vi "CIMfpgaVI.vi"() -> ()   [LabVIEW 2016]
uses:
  Controls/StatesCIM.ctl
  Controls/srcmODE.ctl
  <vilib>/rvi/eio/common/nirviEmuClasses.ctl
  <vilib>/rvi/Emulation/niFpgaGetClockAttributes.vi
  <vilib>/rvi/Emulation/niFpgaSctlEmulationGetInTimedLoop.vi
  <vilib>/rvi/Emulation/niFpgaEmulationReportErrorSimple.vi
  <vilib>/rvi/Emulation/niFpgaProcessEmulError.vi
  <vilib>/rvi/Emulation/niFpgaCriticalErrorInLSC.vi
  <vilib>/rvi/occurrence/nirviWaitOnOccurrenceBase.vi
  <vilib>/rvi/Emulation/niFpgaEmulationIsFPGAContextNoSignature.vi
  <vilib>/rvi/errors/niFpgaSetErrorForExecOnDevCompSimple.vi
  <vilib>/rvi/eio/common/nirviEmuReportErrorAndStop.vi
  <vilib>/rvi/DataTransferAndStorage/Container/Common/niFpgaContainerGetUniqueNameForEmu.vi
  <vilib>/rvi/FIFO/Fifo_Resource/nirvififoEmulationSetSize.vi
  <vilib>/rvi/FIFO/Fifo_Resource/nirviFifoEmulationQueueMgr.vi
  <instcachedir>/0/nirviFifoEmulationQueueMgr_E5CAEC123FF24DC58D834DCA3CDAA9B5.lvgen/nirviFifoEmulationQueueMgr_E5CAEC123FF24DC58D834DCA3CDAA9B5_002.vi
  <vilib>/Utility/error.llb/Clear Errors.vi
  <vilib>/rvi/FIFO/Fifo_Resource/nirvififoEmulationCreateLock.vi
  <vilib>/rvi/FIFO/Fifo_Resource/nirvififoEmulationObtainLock.vi
  <vilib>/rvi/FIFO/Fifo_Resource/nirvififoEmulationReleaseLock.vi
  <vilib>/rvi/errors/nirviReportUnexpectedCaseInternalError.vi
  <vilib>/rvi/errors/nirviReportUnexpectedCaseInternalError (U32).vi
  <vilib>/rvi/eio/common/nirviEmuTemplateMethod_noerrors.vi
  <vilib>/rvi/eio/common/nirviEmuTemplateMethod_errors.vi
  <instcachedir>/0/nirviFifoEmulationQueueMgr_E5CAEC123FF24DC58D834DCA3CDAA9B5.lvgen/nirviFifoEmulationQueueMgr_E5CAEC123FF24DC58D834DCA3CDAA9B5_001.vi
  <vilib>/rvi/FIFO/Fifo_Resource/nirvififoEmulationDetermineInputValidOut.vi
  <vilib>/rvi/eio/common/nirviEmuTemplatePropertyGet_errors.vi
  <vilib>/rvi/Memory/Memory_Emulation/niFpgaMemoryEmulationCacheClearOnFirstRun.vi
  <vilib>/rvi/Memory/Memory_Emulation/nirvimemoryEmulationManagerCache_MakeExclusive.vi
  <vilib>/rvi/Memory/Memory_Emulation/niFpgaMemoryEmulationValidateCache.vi
  <vilib>/rvi/Memory/Memory_Emulation/nirvimemoryEmulationManagerCache_InsertValue.vi
  <vilib>/rvi/Memory/Memory_Emulation/nirvimemoryEmulationManagerCache_ReleaseExclusive.vi
  <vilib>/rvi/Memory/Memory_Emulation/nirvimemoryEmulationManagerCache_GetValue.vi
  <vilib>/rvi/Memory/Memory_Emulation/nirvimemoryEmulationManagerCache_SetValue.vi
  <vilib>/rvi/DataTransferAndStorage/Container/XNode/niFpgaContainer.xnode
  <vilib>/rvi/FIFO/Fifo_Resource/nirvififoEmulationRead.vi
  <vilib>/rvi/FXPMathLib/FxpMul/XNode/nifxpmath_Multiplier.xnode
  <vilib>/eio/EIOGrowableMethodNode/genericMethod/EIOGrowableMethodNode.xnode
  <vilib>/rvi/eio/nirviEIOMethodImplementation/nirviEIOMethodImplementation.xnode
  <vilib>/rvi/eio/nirviErrorMerge/nirviErrorMerge.xnode
  <vilib>/rvi/FIFO/Fifo_Resource/nirvififoEmulationWrite.vi
  <vilib>/eio/EIONode/EIONode.xnode
  <vilib>/eio/EIOPropertyNode/EIOPropertyNode.xnode
  <vilib>/eio/EIOMethodNode/EIOMethodNode.xnode
  <vilib>/rvi/DataTransferAndStorage/Register/Emulation/niFpgaRegisterEmulation.vi
  <vilib>/rvi/eio/common/nirviEmuTemplatePropertyGet_noerrors.vi
  <vilib>/rvi/eio/common/nirviEmuTemplatePropertySet_errors.vi
  <vilib>/rvi/eio/common/nirviEmuTemplatePropertySet_noerrors.vi
  <vilib>/rvi/FXPMathLib/sim/FxpSim.dll
panel:
  out "State Set":T1
  out "ACCT current":fxp<+/-,24,5>
  out "Vmon current":fxp<+/-,24,5>
  out "ACCTThr_readback":fxp<+/-,24,5>=5.5
  out "VMONThr_readback":fxp<+/-,24,5>=-3.0
  out "VMONOff_readback":fxp<+/-,24,5>=-1.0
  out "DUTY Bad Cycles":u32
  out "acct gateon":fxp<+/-,24,5>
  out "vmon gateon":fxp<+/-,24,5>
  out "Modules error":errorcluster
  out "State Diag":T1
  out "VMon Diag":fxp<+/-,24,5>
  out "ACCT Diag":fxp<+/-,24,5>
  out "FBIs":u32
  out "Faraday Diag":bool
  out "C.GATE Diag":bool
  out "Duty Diag":bool=TRUE
  out "Pulse Diag":bool=TRUE
  out "AQ DI24V 2":u32
  out "DI24V LOOP TICKS":u8 caption="Data loop time (usec)"
  out "Timed Out? 5":bool
  out "Timed Out? 6":bool
  out "Timed Out? 7":bool
  in  "DI24V timeout":i32=40
  in  "DI24V sample period (ticks)":u32=40
  out "SRCDuty":fxp<+,32,32>=20.0
  out "SRCPulse":u32=120200
  out "SRCMode":T2
  in  "RESET":bool
  in  "TTL sample period (ticks)":u32=20
  in  "TTL timeout":i32=40
  out "ANALOG LOOP TICKS 2":u8 caption="Data loop time (usec)"
  out "DITTL LOOP TICKS":u8 caption="Data loop time (usec)"
  out "FBI LOOP TICKS":u8 caption="Data loop time (usec)"
  out "Timed Out? 10":bool
  out "Timed Out? 9":bool
  out "DUTY Loop time (tick)":u32
  out "acct gateoff":fxp<+/-,24,5>
  out "Vmon gateoff":fxp<+/-,24,5>
  out "chopper gate":bool
  out "Faraday":bool
  out "chopper OK":bool
  out "acct prearm":fxp<+/-,24,5>
  out "vmon prearm":fxp<+/-,24,5>
  out "STM Loop time (tick)":u32
  out "Timed Out? 8":bool
  out "Timed Out? 2":bool
  out "Timed Out?":bool
  in  "AI sample period (usec)":u32=1
  out "DUTY CYCLING":u32
  out "BULCE AQ GRANDE":i32
  out "DO24V":u32
  out "AQ DITTL":u32
  out "AQ ANALOG STATUS":u32
  out "AQ ANALOG PULSOS":u32
  out "Duty Waiting?":bool
  out "Aquisition Waiting?":bool
  in  "AI Timeout":i32=400
  out "AQ ANALOG AI01":u32
  out "A. READ timeout":bool
  out "current state":T1
  out "State machine iterations":u32
  out "config":i32
  in  "ACCTThr":fxp<+/-,24,5>=5.5
  in  "VMONThr":fxp<+/-,24,5>=-3.0
  in  "GATETFall (us)":u8=15
  in  "GATETRise (us)":u8=15
  in  "VMONOff":fxp<+/-,24,5>=-1.0
  out "FBI":bool
  out "cRIOModulesOK":bool
  out "Mod1Present 4":bool
  out "Mod1Present 3":bool
  out "Mod1Present 2":bool
  out "Mod1Present":bool
  out "Module ID 4":u16
  out "Module ID 3":u16
  out "Module ID 2":u16
  out "Module ID":u16
  out "Duty & Pulse OK?":bool
  out "Low Period (Ticks)":u32
  out "High Period (Ticks)":u32
  out "Pulse OK":bool
  out "Duty OK":bool
  out "Read/write Error":errorcluster
  out "Overwrite":bool
  out "Sample Gated":bool
  in  "StopLoops":bool
  # "System tick is 25ns, \n40 ticks = 1 microsencod (usec)"
  # "ARMED"
  # "CONFIGURATION"
  # "ERROR"
  # "AQ debug"
  # "OPERATION"
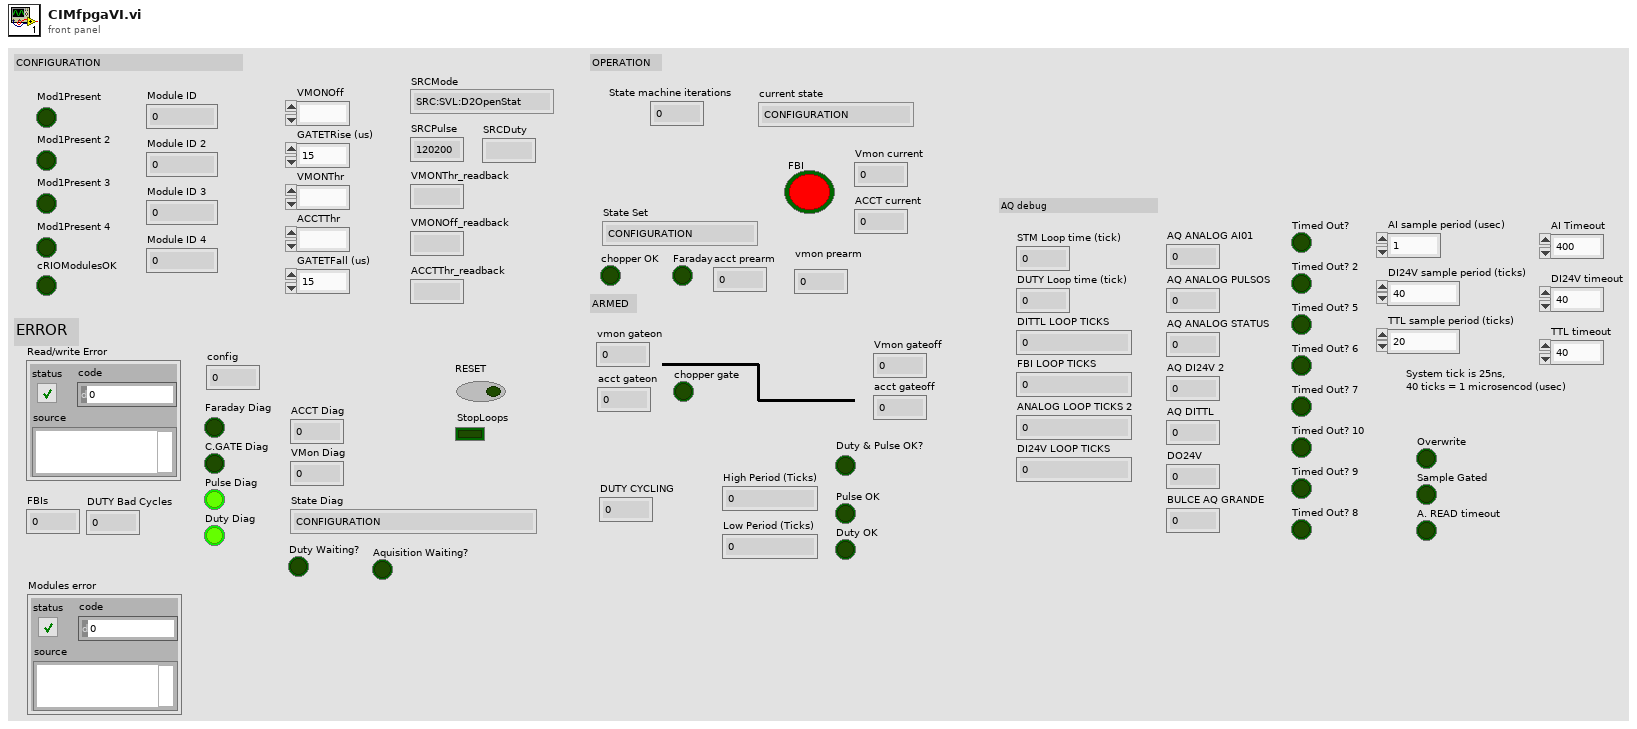
[diagram p1: front panel]
types:
  T1 = typedef "StatesCIM.ctl" = enum16{"CONFIGURATION", "PRE-ARM", "ARMED", "GATE OFF", "GATE ON: RISING", "GATE ON", "GATE OFF: DECREASING"}
  T2 = typedef "srcmODE.ctl" = enum16{"SRC:SVL:D2OpenStat", "SRC:SVL:H2OpenStat"}
  T3 = typedef "nirviEmuClasses.ctl" = enum16{"IO Read", "IO Write", "Method", "Property Read", "Property Write"}
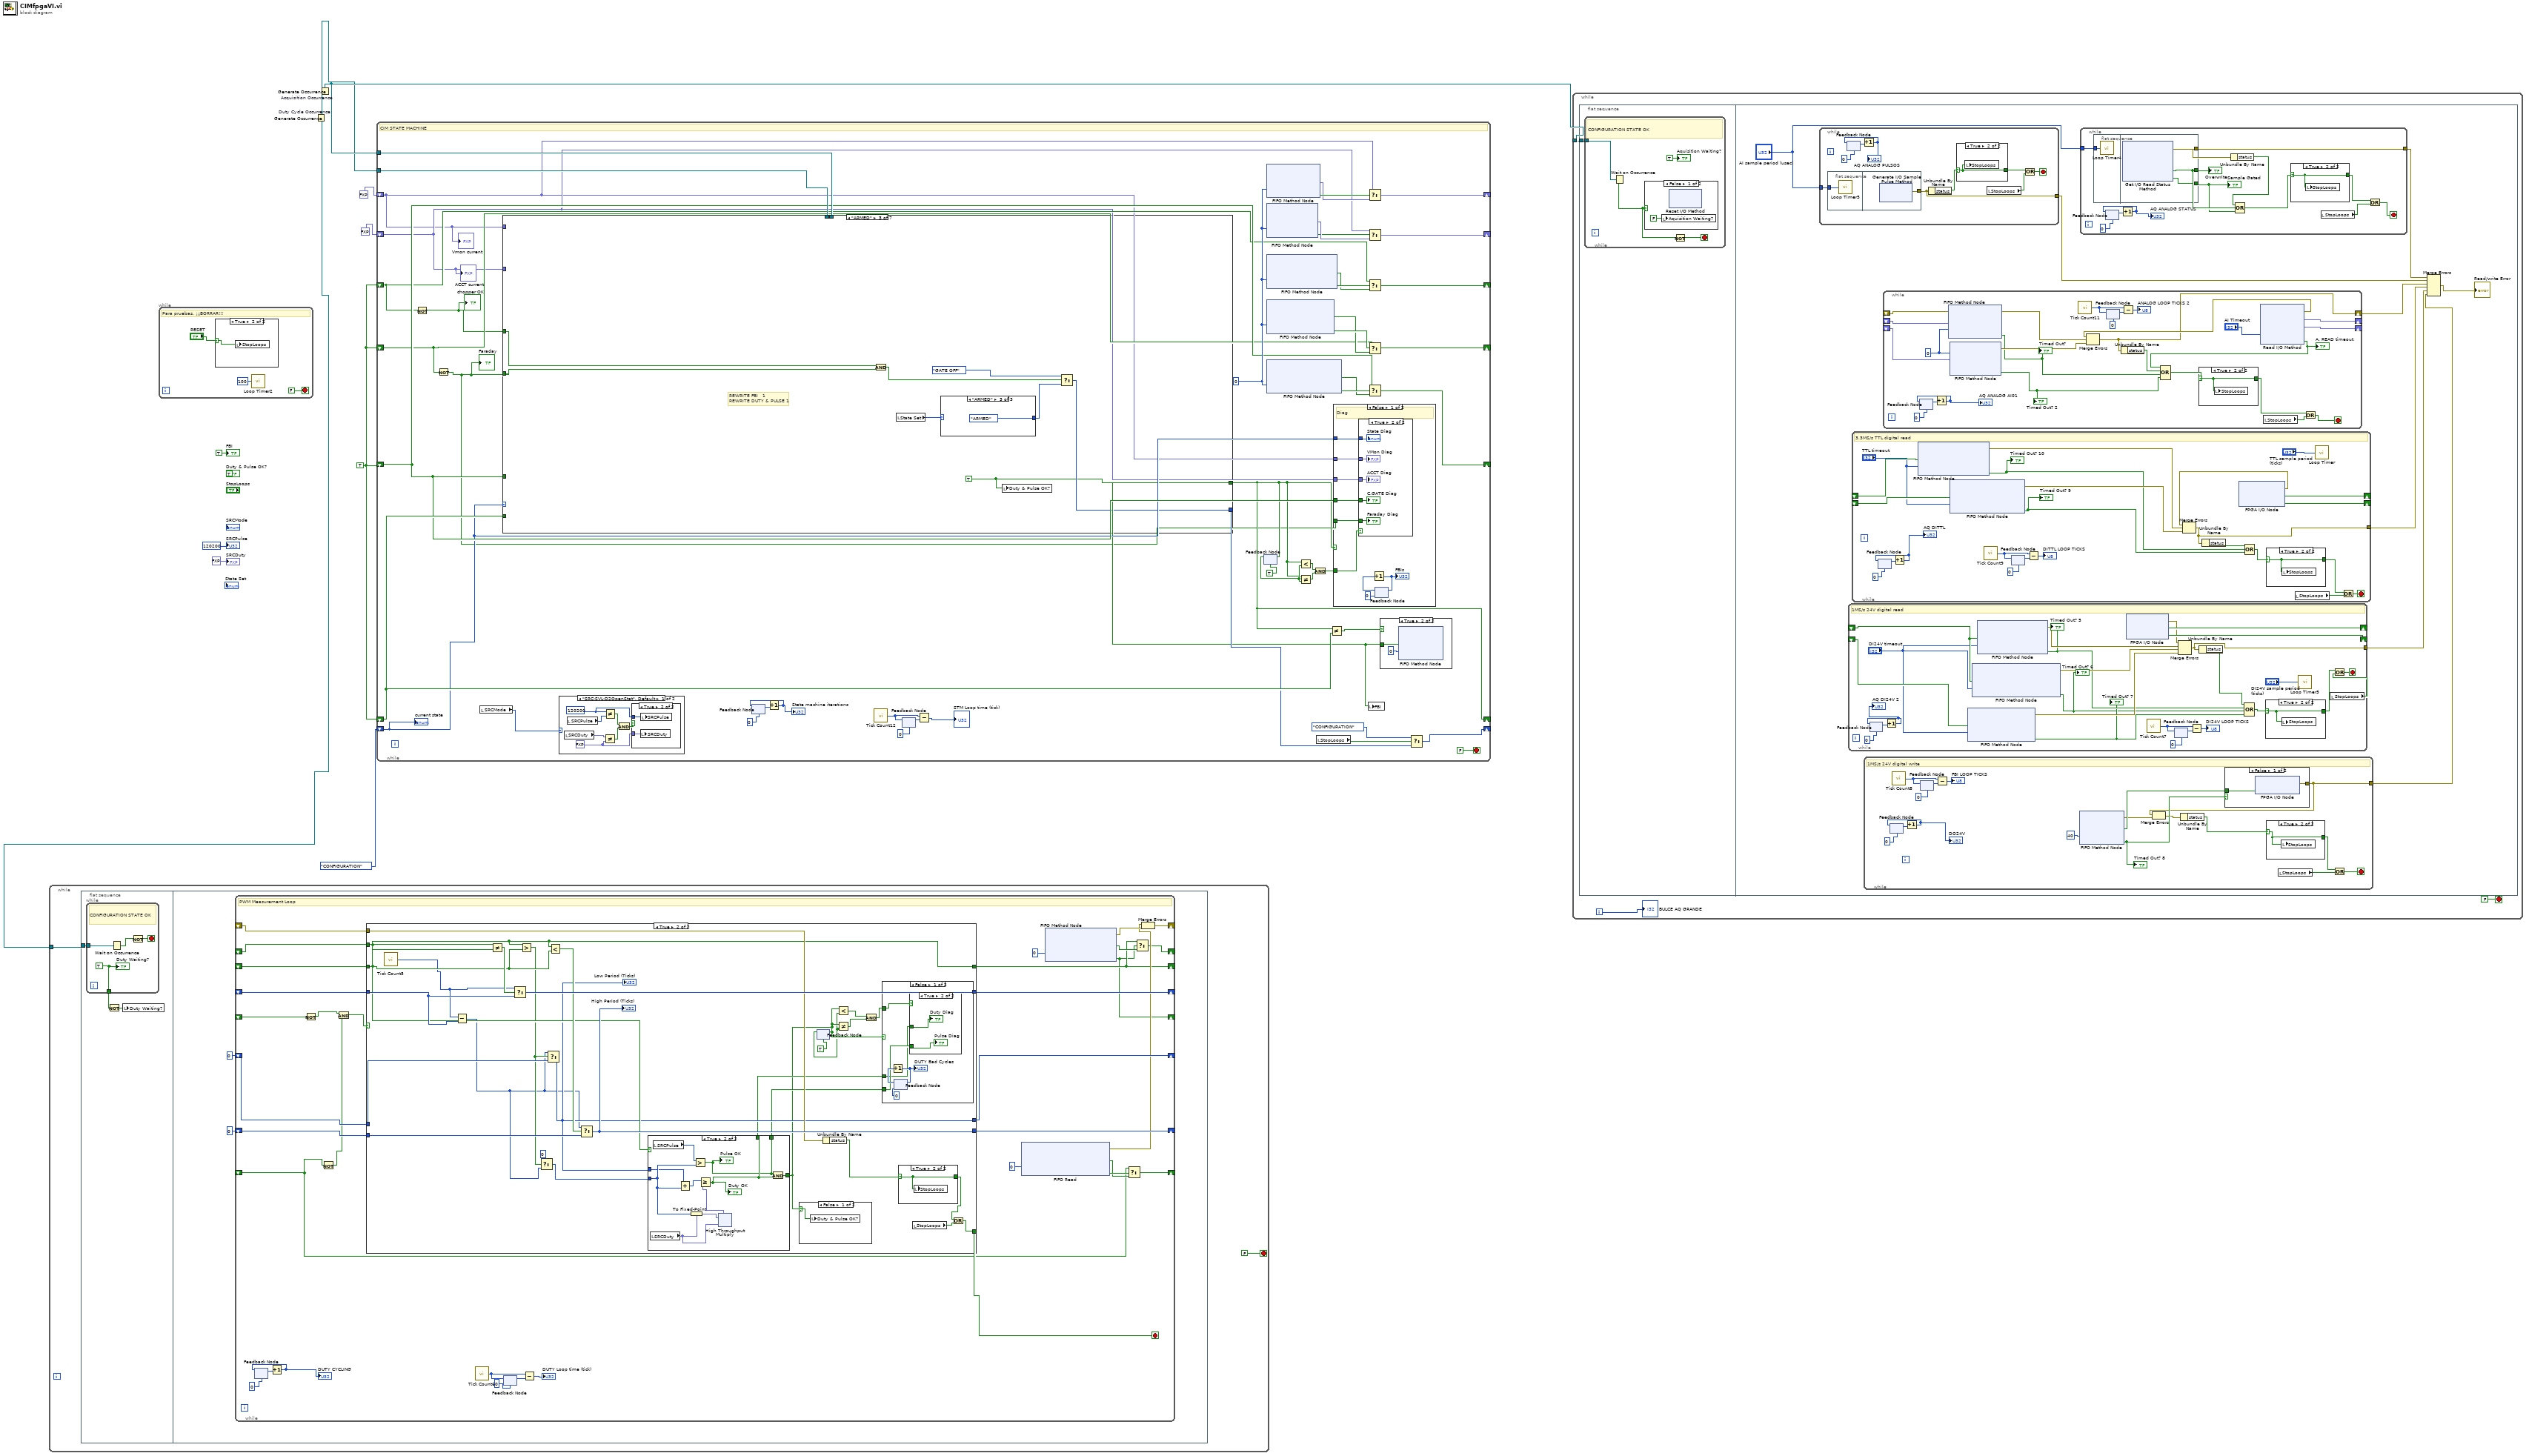
[diagram p0: block diagram]
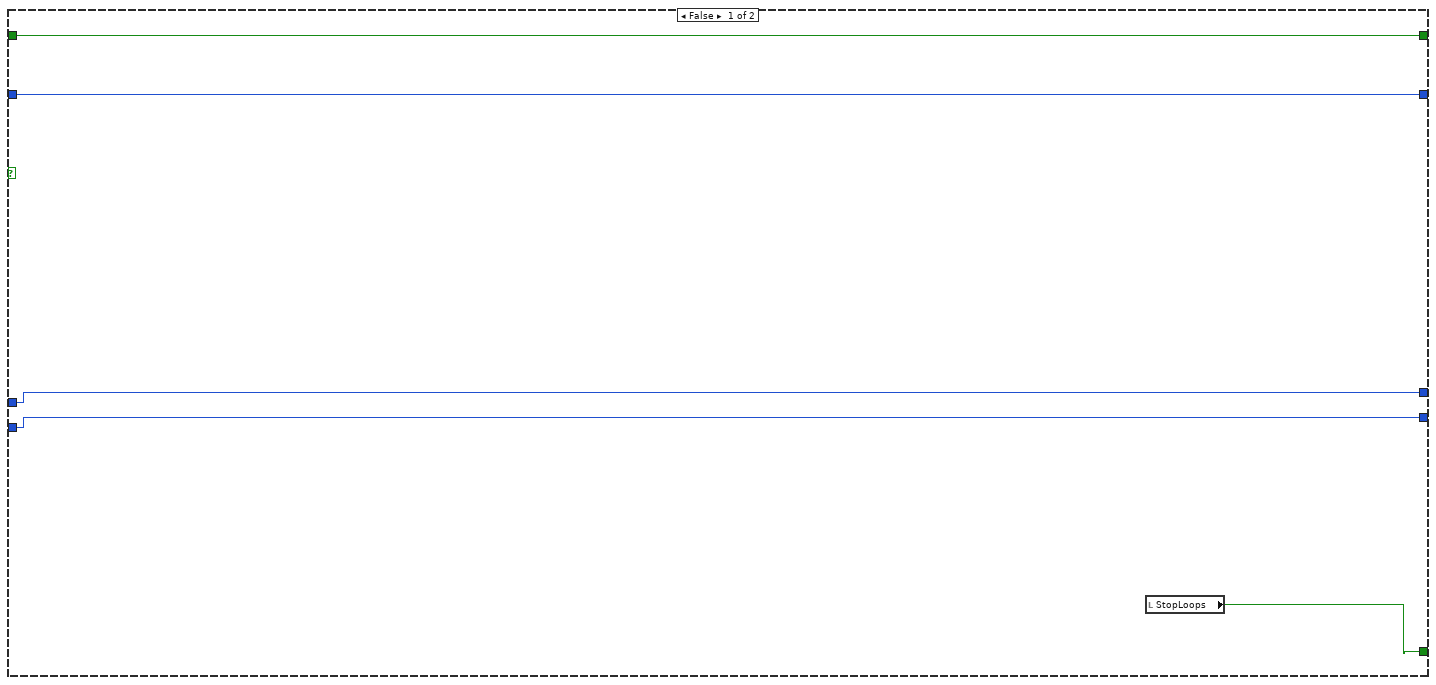
[diagram p2: hidden frame]
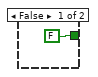
[diagram p6: hidden frame]
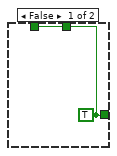
[diagram p7: hidden frame]
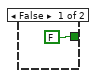
[diagram p10: hidden frame]
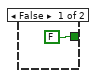
[diagram p11: hidden frame]
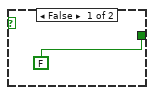
[diagram p12: hidden frame]
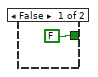
[diagram p14: hidden frame]
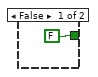
[diagram p15: hidden frame]
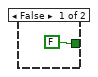
[diagram p16: hidden frame]
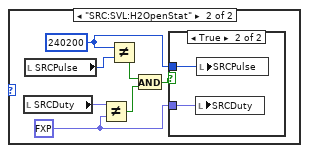
[diagram p18: hidden frame]
diagram:
  w10 = TRUE
  n1 = while {
    stop <- FALSE stop-if-true
    # "Para pruebas. ¡¡¡BORRAR!!!"
    n2 = case shown="True" "RESET" {
      selector: "RESET" -> [_ w14]
      frame False {
      }
      frame True {
        n3 = local write "StopLoops"(w14) -> ()
      }
    }
    n4 = call "Loop Timer2"("Count(mSec)"=u32 100) -> ()  [unwired: 1 out]
  }
  n5 = Generate Occurrence "Duty Cycle Occurrence"() -> (w2:refnum<k4>)
  n6 = while {
    tunnel: w2 -> [w15]
    stop <- FALSE stop-if-true
    n7 = flat-sequence {
      tunnel: w15 -> [w17]
      frame #0 {
        n8 = while {
          tunnel: [w21] -> w19
          tunnel: w17 -> [w20]
          stop <- w22 stop-if-true
          w21 = TRUE ("Duty Waiting?")
          # "CONFIGURATION STATE OK"
          n9 = Wait on Occurrence(2:w20) -> (0:w23:bool)  [unwired: 2 in]
          n10 = Not(x=w23) -> (.not. x?=w22:bool)
          "Duty Waiting?" <- w21
        }
        n11 = Not(x=w19) -> (.not. x?=w18:bool)
        n12 = local write "Duty Waiting?"(w18) -> ()
      }
      frame #1 {
        n13 = while {
          shift-left: u32 0 -> [w58]
          shift-right: [w54] -> _
          shift-left: u32 0 -> [w55]
          shift-right: [w52] -> _
          shift-left: _ -> [w59]
          shift-right: [w45] -> _
          shift-left: _ -> [w56]
          shift-right: [w57] -> _
          shift-right: [w48] -> _
          shift-left: _ -> [w27]
          shift-right: [w44] -> _
          shift-left: _ -> [w43]
          shift-right: [w42] -> _
          shift-left: _ -> [w39]
          shift-right: [w32] -> _
          shift-left: _ -> [w31]
          stop <- w37 stop-if-true
          # "PWM Measurement Loop"
          n14 = feedback #1(u32 0 ("State machine iterations")) -> (w29:u32)
          n15 = Increment(x=w29) -> (x+1=w28:u32)
          "DUTY CYCLING" <- w28
          n16 = feedback-in #1(w28) -> ()
          n17 = Not(x=w39) -> (.not. x?=w38:bool)
          n18 = Not(x=w27) -> (.not. x?=w26:bool)
          n19 = And(x=w38, y=w26) -> (x .and. y?=w40:bool)
          n20 = case shown="True" w40 {
            tunnel: w59 -> [w64 w84]
            tunnel: w58 -> [w61 w91]
            tunnel: [w63 w90] -> w57
            tunnel: w56 -> [w63 w89]
            tunnel: w55 -> [w62 w87]
            tunnel: [w61 w86] -> w54
            tunnel: [w62 w81] -> w52
            tunnel: w31 -> [_ w85]
            tunnel: [w64 w82] -> w45
            tunnel: w43 -> [_ w82]
            tunnel: [w60 w76] -> w37
            frame False {
              n21 = local read "StopLoops"() -> (w60:bool)
            }
            frame True {
              n22 = call "Tick Count5"() -> ("Tick Count(Ticks)"=w83:u32)
              n23 = Subtract(x=w83, y=w89) -> (x-y=w79:u32)
              n24 = Not Equal?(x=w82, y=w84) -> (x != y?=w92:bool)
              n25 = Select(t=w83, s=w92, f=w89) -> (s? t:f=w90:u32)
              n26 = Greater?(x=w82, y=w84) -> (0:w80:bool)
              n27 = Select(t=u32 0, s=w80, f=w79) -> (s? t:f=w78:u32)
              n28 = Select(t=w79, s=w80, f=w87) -> (s? t:f=w81:u32)
              "Low Period (Ticks)" <- w81
              n29 = Less?(x=w82, y=w84) -> (x < y?=w88:bool)
              n30 = Select(t=w79, s=w88, f=w91) -> (s? t:f=w86:u32)
              "High Period (Ticks)" <- w86
              n31 = case shown="True" w82 {
                tunnel: w78 -> [_ w111]
                tunnel: w81 -> [_ w110]
                tunnel: [w104 w109] -> w66
                tunnel: [w104 w106] -> w71
                tunnel: [w104 w105] -> w72
                frame False {
                  w104 = TRUE
                }
                frame True {
                  n32 = local read "SRCDuty"() -> (w108:fxp<+,32,32>)
                  n33 = local read "SRCPulse"() -> (w107:u32)
                  n34 = Add(x=w110, y=w111) -> (x+y=w114:u32)
                  n35 = To Fixed-Point(fixed-point type=w108, number=w111) -> (fixed-point=w112:fxp<+,32,32>)
                  n36 = Greater?(x=w107, y=w111) -> (0:w105:bool)
                  "Pulse OK" <- w105
                  n37 = xnode ("High Throughput Multiply")("x"=w112, "y"=w108) -> ("x*y"=w113:fxp<+,64,64>)
                  n38 = Greater Or Equal?(x=w114, y=w113) -> (x >= y?=w106:bool)
                  "Duty OK" <- w106
                  n39 = And(x=w105, y=w106) -> (x .and. y?=w109:bool)
                }
              }
              n40 = case shown="False" w66 {
                selector: w66 -> [w101 _]
                frame False {
                  n41 = local write "Duty & Pulse OK?"(w101) -> ()
                }
                frame True {
                }
              }
              n42 = feedback #2(TRUE) -> (w65:bool)
              n43 = feedback-in #2(w66) -> ()
              n44 = Unbundle By Name(w85) -> ("status"=w73:bool)
              n45 = Less?(x=w66, y=w65) -> (x < y?=w68:bool)
              n46 = Not Equal?(x=w66, y=w65) -> (x != y?=w69:bool)
              n47 = And(x=w68, y=w69) -> (x .and. y?=w67:bool)
              n48 = case shown="False" w66 {
                tunnel: w72 -> [w95 _]
                tunnel: w71 -> [w94 _]
                tunnel: w67 -> [w93 _]
                frame False {
                  n49 = feedback #3(u32 0) -> (w97:u32)
                  n50 = Increment(x=w97) -> (x+1=w96:u32)
                  "DUTY Bad Cycles" <- w96
                  n51 = feedback-in #3(w96) -> ()
                  n52 = case shown="True" w93 {
                    tunnel: w95 -> [_ w99]
                    tunnel: w94 -> [_ w100]
                    frame False {
                    }
                    frame True {
                      "Duty Diag" <- w100
                      "Pulse Diag" <- w99
                    }
                  }
                }
                frame True {
                }
              }
              n53 = case shown="True" w73 {
                selector: w73 -> [_ w103]
                tunnel: [FALSE w103] -> w75
                frame False {
                }
                frame True {
                  n54 = local write "StopLoops"(w103) -> ()
                }
              }
              n55 = local read "StopLoops"() -> (w74:bool)
              n56 = Or(x=w75, y=w74) -> (x .or. y?=w76:bool)
            }
          }
          n57 = call "Tick Count6"() -> ("Tick Count(Ticks)"=w35:u32)
          n58 = feedback #4(u32 0 ("Tick Count(Ticks)")) -> (w36:u32)
          n59 = feedback-in #4(w35) -> ()
          n60 = Subtract(x=w35, y=w36) -> (x-y=→"DUTY Loop time (tick)":u32)
          n61 = xnode ("FIFO Read")("Timeout"=0) -> ("Element"=w49:bool, "Timed Out?"=w50:bool, "error out"=w46:errorcluster)  [unwired: 2 in, 1 out]
          n62 = xnode ("FIFO Method Node")("Timeout"=0) -> ("Element"=w51:bool, "Timed Out?"=w42:bool, "error out"=w47:errorcluster)  [unwired: 2 in, 1 out]
          n63 = Select(t=w27, s=w50, f=w49) -> (s? t:f=w48:bool)
          n64 = Select(t=w45, s=w42, f=w51) -> (s? t:f=w44:bool)
          n65 = Merge Errors(w46, w47) -> (w32:errorcluster)
        }
      }
    }
  }
  n66 = Generate Occurrence "Acquisition Occurrence"() -> (w6:refnum<k4>)
  n67 = while {
    shift-right: [w135] -> _
    shift-left: StatesCIM."CONFIGURATION" ("STATES") -> [w128]
    shift-right: [w120] -> _
    shift-left: w10 -> [w144]
    shift-right: [w157] -> _
    shift-left: fxp<+/-,24,5> 0.0 ("Element") -> [w115]
    shift-right: [w154] -> _
    shift-left: fxp<+/-,24,5> 0.0 ("Element") -> [w116]
    shift-right: [w146] -> _
    shift-left: w10 -> [w127]
    shift-right: [w145] -> _
    shift-left: w10 -> [w126]
    shift-right: [w150] -> _
    shift-left: w10 -> [w133]
    tunnel: w2 -> [w138]
    tunnel: w6 -> [w137]
    stop <- FALSE stop-if-true
    w160 = 0 ("Timeout")
    # "CIM STATE MACHINE"
    n68 = Not(x=w127) -> (.not. x?=w118:bool)
    "chopper OK" <- w118
    n69 = Not(x=w126) -> (.not. x?=w117:bool)
    "Faraday" <- w117
    n70 = local read "SRCMode"() -> (w119:T2)
    n71 = case shown="\"ARMED\"" w128 {
      tunnel: [w198 w238 w258 w280 w298 w305 w331] -> w132
      tunnel: w144 -> [_ w247 _ _ _ _ _]
      tunnel: [TRUE ("Init done") w247 w257 w271 w296 w308 w326] -> w120
      tunnel: w115 -> [_ w250 _ w267 _ w312 _]
      tunnel: w116 -> [_ w249 _ w278 _ w303 _]
      tunnel: w118 -> [_ _ w261 w269 w293 w310 w329]
      tunnel: w117 -> [_ _ w260 w270 w294 w311 w328]
      tunnel: w133 -> [_ w248 _ w274 w295 w313 w333]
      tunnel: w137 -> [w197 _ _ _ _ _ _]
      tunnel: w138 -> [w196 _ _ _ _ _ _]
      frame "CONFIGURATION", Default {
        n72 = while {
          tunnel: [w220] -> w200
          i -> [w225]
          stop <- w220 stop-if-true
          w234 = refnum<k21> "Mod4"  # cRIO I/O Device
          w235 = refnum<k21> "Mod3"  # cRIO I/O Device
          w236 = refnum<k21> "Mod2"  # cRIO I/O Device
          w237 = refnum<k21> "Mod1"  # cRIO I/O Device
          # "CONFIGURATION"
          n73 = xnode "FPGA I/O Property Node"("FPGA I/O In"=w237) -> ("Module ID"=w227:u16)  [unwired: 1 in, 2 out]
          "Module ID" <- w227
          n74 = xnode "FPGA I/O Property Node"("FPGA I/O In"=w236) -> ("Module ID"=w229:u16)  [unwired: 1 in, 2 out]
          "Module ID 2" <- w229
          n75 = xnode "FPGA I/O Property Node"("FPGA I/O In"=w235) -> ("Module ID"=w231:u16)  [unwired: 1 in, 2 out]
          "Module ID 3" <- w231
          n76 = xnode "FPGA I/O Property Node"("FPGA I/O In"=w234) -> ("Module ID"=w233:u16)  [unwired: 1 in, 2 out]
          "Module ID 4" <- w233
          n77 = Equal?(x=u16 30516 ("Module ID"), y=w227) -> (x = y?=w224:bool)
          "Mod1Present" <- w224
          n78 = Equal?(x=u16 28976 ("Module ID 2"), y=w229) -> (x = y?=w223:bool)
          "Mod1Present 2" <- w223
          n79 = Equal?(x=u16 29130 ("Module ID 3"), y=w231) -> (x = y?=w222:bool)
          "Mod1Present 3" <- w222
          n80 = Equal?(x=u16 28832 ("Module ID 4"), y=w233) -> (x = y?=w221:bool)
          "Mod1Present 4" <- w221
          n81 = Compound Arithmetic op=AND(w224, w223, w222, w221) -> (w220:bool)
          "cRIOModulesOK" <- w220
          "config" <- w225
        }
        n82 = stacked-sequence {
          tunnel: w200 -> [_ _ _]
          tunnel: [_ _ StatesCIM."PRE-ARM" ("STATES")] -> w198
          tunnel: w197 -> [_ _ w219]
          tunnel: w196 -> [_ _ w218]
          tunnel: [_ _ w215] -> _
          frame #0 {
            # "9401 CONFIG"
            n83 = call "Wait2"("Count(mSec)"=u32 1000) -> ()  [unwired: 1 out]
            n84 = xnode "FPGA I/O Method Node"("DIO 7:4"=enum8{"No Change", "Input", "Output"}."Input" ("DIO 3:0"), "DIO 3:0"=enum8{"No Change", "Input", "Output"}."Input") -> ("error out"=w202:errorcluster)  [unwired: 2 in, 1 out]
            n85 = while {
              tunnel: w202 -> [w209]
              stop <- w210 stop-if-true
              n86 = xnode "FPGA I/O Method Node"("error in"=w209) -> ("error out"=w206:errorcluster, "Ready"=w213:bool)  [unwired: 1 in, 1 out]
              n87 = xnode "FPGA I/O Method Node"("error in"=w209) -> ("error out"=w207:errorcluster, "Ready"=w212:bool)  [unwired: 1 in, 1 out]
              n88 = xnode "FPGA I/O Method Node"("error in"=w209) -> ("error out"=w208:errorcluster, "Ready"=w211:bool)  [unwired: 1 in, 1 out]
              n89 = Merge Errors(w206, w207, w208) -> (→"Modules error":errorcluster)
              n90 = Compound Arithmetic op=AND(w213, w212, w211) -> (w210:bool)
            }
          }
          frame #1 {
            n91 = local write "StopLoops"(FALSE ("StopLoops")) -> ()
          }
          frame #2 {
            n92 = Set Occurrence "Set Duty Cycle Occurrence"(w218) -> ()
            n93 = Set Occurrence "Set Acquisition Occurrence"(w219) -> ()
            n94 = xnode "FPGA I/O Node"("Mod4/DO0"=TRUE) -> ("error out"=w215:errorcluster)  [unwired: 2 in, 1 out]
          }
        }
      }
      frame "PRE-ARM" {
        n95 = local read "State Set"() -> (w239:T1)
        n96 = case shown="\"ARMED\"" w239 {
          tunnel: [StatesCIM."PRE-ARM" ("Enum") StatesCIM."PRE-ARM" ("Enum") StatesCIM."ARMED" ("Enum")] -> w238
          frame "CONFIGURATION", Default {
          }
          frame "PRE-ARM" {
          }
          frame "ARMED" {
          }
        }
        n97 = xnode ("Register Write")("Data"="VMONOff") -> ()  [unwired: 1 in, 1 out]
        n98 = xnode ("Register Write")("Data"="VMONThr") -> ()  [unwired: 1 in, 1 out]
        n99 = xnode ("Register Write")("Data"="ACCTThr") -> ()  [unwired: 1 in, 1 out]
        n100 = Increment(x="GATETFall (us)") -> (x+1=w240:u8)
        n101 = Increment(x="GATETRise (us)") -> (x+1=w241:u8)
        n102 = xnode ("Register Write")("Data"=w241) -> ()  [unwired: 1 in, 1 out]
        n103 = xnode ("Register Write")("Data"=w240) -> ()  [unwired: 1 in, 1 out]
        "vmon prearm" <- w250
        "acct prearm" <- w249
        "chopper gate" <- w248
        "VMONOff_readback" <- "VMONOff"
        "VMONThr_readback" <- "VMONThr"
        "ACCTThr_readback" <- "ACCTThr"
      }
      frame "ARMED" {
        w257 = TRUE
        # "REWRITE FBI   1\nREWRITE DUTY & PULSE 1"
        n104 = And(x=w261, y=w260) -> (x .and. y?=w254:bool)
        n105 = local read "State Set"() -> (w256:T1)
        n106 = case shown="\"ARMED\"" w256 {
          tunnel: [StatesCIM."ARMED" ("Enum") StatesCIM."PRE-ARM" ("Enum") StatesCIM."ARMED" ("Enum")] -> w255
          frame "CONFIGURATION", Default {
          }
          frame "PRE-ARM" {
          }
          frame "ARMED" {
          }
        }
        n107 = local write "Duty & Pulse OK?"(w257) -> ()
        n108 = Select(t=StatesCIM."GATE OFF" ("Enum"), s=w254, f=w255) -> (s? t:f=w258:T1)
      }
      frame "GATE OFF" {
        # "IF FARADAY=\"0\" AND CHOPPER_GATE=\"0\" TRANSITION INTO PRE-ARM."
        n109 = xnode ("Register Read")() -> ("Data"=w277:fxp<+/-,24,5>)  [unwired: 1 in, 1 out]
        n110 = xnode ("Register Read")() -> ("Data"=w268:fxp<+/-,24,5>)  [unwired: 1 in, 1 out]
        n111 = Greater?(x=w277, y=w278) -> (0:w276:bool)
        n112 = Less?(x=w268, y=w267) -> (x < y?=w266:bool)
        n113 = local read "Duty & Pulse OK?"() -> (w275:bool)
        n114 = case shown="True" w274 {
          selector: w274 -> [w283 w285]
          tunnel: [StatesCIM."GATE OFF" ("Enum") StatesCIM."GATE ON: RISING" ("Enum")] -> w279
          tunnel: [w283 w285] -> w273
          frame False {
          }
          frame True {
            n115 = call "Tick Count"() -> ("Tick Count(uSec)"=w286:u8)
            n116 = xnode ("Register Write")("Data"=w286) -> ()  [unwired: 1 in, 1 out]
          }
        }
        n117 = Compound Arithmetic op=AND(w269, w266, w276, w270, w275) -> (w265:bool)
        n118 = case shown="False" w265 {
          frame False {
            n119 = local write "State Set"(StatesCIM."CONFIGURATION" ("Enum")) -> ()
          }
          frame True {
          }
        }
        n120 = Not Or(1:w270, 2:w273) -> (0:w272:bool)
        n121 = Select(t=w279, s=w265, f=StatesCIM."PRE-ARM" ("Enum")) -> (s? t:f=w280:T1)
        n122 = Or(x=w272, y=w265) -> (x .or. y?=w271:bool)
        "Vmon gateoff" <- w267
        "acct gateoff" <- w278
      }
      frame "GATE ON: RISING" {
        n123 = xnode ("Register Read")() -> ("Data"=w291:u8)  [unwired: 1 in, 1 out]
        n124 = call "Tick Count2"() -> ("Tick Count(uSec)"=w292:u8)
        n125 = xnode ("Register Read")() -> ("Data"=w289:u8)  [unwired: 1 in, 1 out]
        n126 = Subtract(x=w292, y=w291) -> (x-y=w290:u8)
        n127 = Greater Or Equal?(x=w290, y=w289) -> (x >= y?=w300:bool)
        n128 = local read "Duty & Pulse OK?"() -> (w288:bool)
        n129 = case shown="True" w300 {
          tunnel: [StatesCIM."GATE ON: RISING" ("Enum") StatesCIM."GATE ON" ("Enum")] -> w297
          frame False {
          }
          frame True {
          }
        }
        n130 = Compound Arithmetic op=AND(w293, w294, w295, w288) -> (w296:bool)
        n131 = Select(t=w297, s=w296, f=StatesCIM."PRE-ARM" ("Enum")) -> (s? t:f=w298:T1)
      }
      frame "GATE ON" {
        n132 = case shown="True" w313 {
          tunnel: [StatesCIM."GATE OFF: DECREASING" ("Enum") StatesCIM."GATE ON" ("Enum")] -> w306
          tunnel: w312 -> [_ w319]
          tunnel: [TRUE w317] -> w309
          frame False {
            n133 = call "Tick Count3"() -> ("Tick Count(uSec)"=w315:u8)
            n134 = xnode ("Register Write")("Data"=w315) -> ()  [unwired: 1 in, 1 out]
          }
          frame True {
            n135 = xnode ("Register Read")() -> ("Data"=w318:fxp<+/-,24,5>)  [unwired: 1 in, 1 out]
            n136 = Less?(x=w319, y=w318) -> (x < y?=w317:bool)
          }
        }
        n137 = local read "Duty & Pulse OK?"() -> (w304:bool)
        n138 = Compound Arithmetic op=AND(w309, w310, w311, w304) -> (w308:bool)
        n139 = Select(t=w306, s=w308, f=StatesCIM."PRE-ARM" ("Enum")) -> (s? t:f=w305:T1)
        "vmon gateon" <- w312
        "acct gateon" <- w303
      }
      frame "GATE OFF: DECREASING" {
        n140 = xnode ("Register Read")() -> ("Data"=w324:u8)  [unwired: 1 in, 1 out]
        n141 = call "Tick Count4"() -> ("Tick Count(uSec)"=w325:u8)
        n142 = xnode ("Register Read")() -> ("Data"=w322:u8)  [unwired: 1 in, 1 out]
        n143 = Not(x=w333) -> (.not. x?=w327:bool)
        n144 = Subtract(x=w325, y=w324) -> (x-y=w323:u8)
        n145 = local read "Duty & Pulse OK?"() -> (w321:bool)
        n146 = Greater Or Equal?(x=w323, y=w322) -> (x >= y?=w334:bool)
        n147 = case shown="True" w334 {
          tunnel: [StatesCIM."GATE OFF: DECREASING" ("Enum") StatesCIM."GATE OFF" ("Enum")] -> w330
          frame False {
          }
          frame True {
          }
        }
        n148 = Compound Arithmetic op=AND(w329, w328, w327, w321) -> (w326:bool)
        n149 = Select(t=w330, s=w326, f=StatesCIM."PRE-ARM" ("Enum")) -> (s? t:f=w331:T1)
      }
    }
    n150 = case shown="\"SRC:SVL:D2OpenStat\", Default" w119 {
      frame "SRC:SVL:D2OpenStat", Default {
        w163 = fxp<+,32,32> 20.0 ("maxDuty")
        w164 = u32 120200 ("maxHigh")
        n151 = local read "SRCDuty"() -> (w168:fxp<+,32,32>)
        n152 = local read "SRCPulse"() -> (w167:u32)
        n153 = Not Equal?(x=w168, y=w163) -> (x != y?=w165:bool)
        n154 = Not Equal?(x=w164, y=w167) -> (x != y?=w166:bool)
        n155 = And(x=w166, y=w165) -> (x .and. y?=w162:bool)
        n156 = case shown="True" w162 {
          tunnel: w164 -> [_ w170]
          tunnel: w163 -> [_ w169]
          frame False {
          }
          frame True {
            n157 = local write "SRCDuty"(w169) -> ()
            n158 = local write "SRCPulse"(w170) -> ()
          }
        }
      }
      frame "SRC:SVL:H2OpenStat" {
        w172 = fxp<+,32,32> 10.0 ("maxDuty")
        w171 = u32 240200 ("maxHigh")
        n159 = local read "SRCDuty"() -> (w177:fxp<+,32,32>)
        n160 = local read "SRCPulse"() -> (w176:u32)
        n161 = Not Equal?(x=w177, y=w172) -> (x != y?=w174:bool)
        n162 = Not Equal?(x=w171, y=w176) -> (x != y?=w175:bool)
        n163 = And(x=w175, y=w174) -> (x .and. y?=w173:bool)
        n164 = case shown="True" w173 {
          tunnel: w172 -> [_ w179]
          tunnel: w171 -> [_ w178]
          frame False {
          }
          frame True {
            n165 = local write "SRCDuty"(w179) -> ()
            n166 = local write "SRCPulse"(w178) -> ()
          }
        }
      }
    }
    n167 = feedback #5(u32 0 ("State machine iterations")) -> (w130:u32)
    n168 = Increment(x=w130) -> (x+1=w129:u32)
    "State machine iterations" <- w129
    n169 = feedback-in #5(w129) -> ()
    n170 = call "Tick Count12"() -> ("Tick Count(Ticks)"=w140:u32)
    n171 = feedback #6(u32 0 ("Tick Count(uSec)")) -> (w141:u32)
    n172 = feedback-in #6(w140) -> ()
    n173 = Subtract(x=w140, y=w141) -> (x-y=→"STM Loop time (tick)":u32)
    n174 = feedback #7(TRUE) -> (w121:bool)
    n175 = feedback-in #7(w120) -> ()
    n176 = xnode ("FIFO Method Node")("Timeout"=w160) -> ("Element"=w158:fxp<+/-,24,5>, "Timed Out?"=w159:bool)  [unwired: 2 in, 2 out]
    n177 = xnode ("FIFO Method Node")("Timeout"=w160) -> ("Element"=w156:fxp<+/-,24,5>, "Timed Out?"=w155:bool)  [unwired: 2 in, 2 out]
    n178 = xnode ("FIFO Method Node")("Timeout"=w160) -> ("Element"=w148:bool, "Timed Out?"=w153:bool)  [unwired: 2 in, 2 out]
    n179 = xnode ("FIFO Method Node")("Timeout"=w160) -> ("Element"=w147:bool, "Timed Out?"=w152:bool)  [unwired: 2 in, 2 out]
    n180 = xnode ("FIFO Method Node")("Timeout"=w160) -> ("Element"=w149:bool, "Timed Out?"=w151:bool)  [unwired: 2 in, 2 out]
    n181 = Less?(x=w120, y=w121) -> (x < y?=w124:bool)
    n182 = Not Equal?(x=w120, y=w121) -> (x != y?=w123:bool)
    n183 = And(x=w124, y=w123) -> (x .and. y?=w122:bool)
    n184 = local read "StopLoops"() -> (w136:bool)
    n185 = Not Equal?(x=w120, y=w144) -> (x != y?=w143:bool)
    n186 = case shown="False" w120 {
      tunnel: w117 -> [w185 _]
      tunnel: w133 -> [w184 _]
      tunnel: w116 -> [w183 _]
      tunnel: w115 -> [w182 _]
      tunnel: w128 -> [w181 _]
      tunnel: w122 -> [w180 _]
      frame False {
        # "Diag"
        n187 = case shown="True" w180 {
          tunnel: w185 -> [_ w193]
          tunnel: w184 -> [_ w192]
          tunnel: w183 -> [_ w191]
          tunnel: w182 -> [_ w190]
          tunnel: w181 -> [_ w189]
          frame False {
          }
          frame True {
            "Faraday Diag" <- w193
            "C.GATE Diag" <- w192
            "ACCT Diag" <- w191
            "VMon Diag" <- w190
            "State Diag" <- w189
          }
        }
        n188 = feedback #8(u32 0) -> (w187:u32)
        n189 = Increment(x=w187) -> (x+1=w188:u32)
        "FBIs" <- w188
        n190 = feedback-in #8(w188) -> ()
      }
      frame True {
      }
    }
    n191 = local write "FBI"(w120) -> ()
    n192 = Select(t=w115, s=w159, f=w158) -> (s? t:f=w157:fxp<+/-,24,5>)
    n193 = Select(t=w116, s=w155, f=w156) -> (s? t:f=w154:fxp<+/-,24,5>)
    n194 = Select(t=w127, s=w153, f=w148) -> (s? t:f=w146:bool)
    n195 = Select(t=w126, s=w152, f=w147) -> (s? t:f=w145:bool)
    n196 = Select(t=w133, s=w151, f=w149) -> (s? t:f=w150:bool)
    n197 = case shown="True" w143 {
      tunnel: w120 -> [_ w194]
      frame False {
      }
      frame True {
        n198 = xnode ("FIFO Method Node")("Element"=w194, "Timeout"=0) -> ()  [unwired: 1 in, 2 out]
      }
    }
    n199 = Select(t=StatesCIM."CONFIGURATION", s=w136, f=w132) -> (s? t:f=w135:T1)
    "current state" <- w128
    "Vmon current" <- w115
    "ACCT current" <- w116
  }
  n200 = while {
    tunnel: w6 -> [w337]
    i -> [w339]
    stop <- FALSE stop-if-true
    n201 = flat-sequence {
      tunnel: w337 -> [w340]
      frame #0 {
        n202 = while {
          tunnel: w340 -> [w343]
          stop <- w341 stop-if-true
          # "CONFIGURATION STATE OK"
          n203 = Wait on Occurrence(2:w343) -> (0:w342:bool)  [unwired: 2 in]
          n204 = case shown="False" w342 {
            frame False {
              n205 = local write "Aquisition Waiting?"(FALSE ("Aquisition Ready?")) -> ()
              n206 = xnode "Reset I/O Method"() -> ()  [unwired: 2 in, 2 out]
            }
            frame True {
            }
          }
          n207 = Not(x=w342) -> (.not. x?=w341:bool)
          "Aquisition Waiting?" <- TRUE ("Aquisition Waiting?")
        }
      }
      frame #1 {
        n208 = while {
          tunnel: "AI sample period (usec)" -> [w699]
          tunnel: [w698] -> w357
          stop <- w695 stop-if-true
          n209 = flat-sequence {
            tunnel: w699 -> [w702]
            tunnel: [w703] -> w698
            frame #0 {
              n210 = call "Loop Timer3"("Count(uSec)"=w702) -> ()  [unwired: 1 out]
            }
            frame #1 {
              n211 = xnode "Generate I/O Sample Pulse Method"() -> ("error out"=w703:errorcluster)  [unwired: 2 in, 1 out]
            }
          }
          n212 = feedback #9(u32 0 ("State machine iterations")) -> (w692:u32)
          n213 = Increment(x=w692) -> (x+1=w691:u32)
          "AQ ANALOG PULSOS" <- w691
          n214 = feedback-in #9(w691) -> ()
          n215 = Unbundle By Name(w698) -> ("status"=w697:bool)
          n216 = case shown="True" w697 {
            selector: w697 -> [_ w701]
            tunnel: [FALSE w701] -> w696
            frame False {
            }
            frame True {
              n217 = local write "StopLoops"(w701) -> ()
            }
          }
          n218 = local read "StopLoops"() -> (w694:bool)
          n219 = Or(x=w696, y=w694) -> (x .or. y?=w695:bool)
        }
        n220 = while {
          tunnel: [w372] -> w352
          shift-right: [w381] -> _
          shift-left: _ -> [w375]
          shift-right: [w380] -> _
          shift-left: _ -> [w376]
          stop <- w370 stop-if-true
          # "1MS/s 24V digital read"
          n221 = feedback #10(u32 0 ("State machine iterations")) -> (w361:u32)
          n222 = Increment(x=w361) -> (x+1=w360:u32)
          "AQ DI24V 2" <- w360
          n223 = feedback-in #10(w360) -> ()
          n224 = xnode ("FIFO Method Node")("Element"=w376, "Timeout"="DI24V timeout") -> ("Timed Out?"=w364:bool, "error out"=w377:errorcluster)  [unwired: 2 in, 1 out]
          "Timed Out? 7" <- w364
          n225 = xnode ("FIFO Method Node")("Element"=w375, "Timeout"="DI24V timeout") -> ("Timed Out?"=w363:bool, "error out"=w378:errorcluster)  [unwired: 2 in, 1 out]
          "Timed Out? 6" <- w363
          n226 = xnode ("FIFO Method Node")("Element"=w375, "Timeout"="DI24V timeout") -> ("Timed Out?"=w369:bool, "error out"=w379:errorcluster)  [unwired: 2 in, 1 out]
          "Timed Out? 5" <- w369
          n227 = xnode "FPGA I/O Node"() -> ("error out"=w367:errorcluster, "Mod3/DI0"=w381:bool, "Mod3/DI1"=w380:bool)  [unwired: 3 in, 2 out]
          n228 = call "Tick Count7"() -> ("Tick Count(Ticks)"=w383:u8)
          n229 = feedback #11(u8 0 ("Tick Count(uSec)")) -> (w384:u8)
          n230 = feedback-in #11(w383) -> ()
          n231 = Merge Errors(w367, w379, w378, w377) -> (w372:errorcluster)
          n232 = Subtract(x=w383, y=w384) -> (x-y=→"DI24V LOOP TICKS":u8)
          n233 = Unbundle By Name(w372) -> ("status"=w365:bool)
          n234 = Compound Arithmetic op=OR(w365, w369, w363, w364) -> (w374:bool)
          n235 = case shown="True" w374 {
            selector: w374 -> [_ w387]
            tunnel: [FALSE w387] -> w371
            frame False {
            }
            frame True {
              n236 = local write "StopLoops"(w387) -> ()
            }
          }
          n237 = call "Loop Timer5"("Count(Ticks)"="DI24V sample period (ticks)") -> ()  [unwired: 1 out]
          n238 = local read "StopLoops"() -> (w366:bool)
          n239 = Or(x=w371, y=w366) -> (x .or. y?=w370:bool)
        }
        n240 = while {
          tunnel: [w397] -> w354
          shift-right: [w404] -> _
          shift-left: _ -> [w402]
          shift-right: [w405] -> _
          shift-left: _ -> [w403]
          stop <- w395 stop-if-true
          # "3,3MS/s TTL digital read"
          n241 = feedback #12(u32 0 ("State machine iterations")) -> (w389:u32)
          n242 = Increment(x=w389) -> (x+1=w388:u32)
          "AQ DITTL" <- w388
          n243 = feedback-in #12(w388) -> ()
          n244 = xnode ("FIFO Method Node")("Element"=w403, "Timeout"="TTL timeout") -> ("Timed Out?"=w393:bool, "error out"=w399:errorcluster)  [unwired: 2 in, 1 out]
          "Timed Out? 10" <- w393
          n245 = xnode ("FIFO Method Node")("Element"=w402, "Timeout"="TTL timeout") -> ("Timed Out?"=w392:bool, "error out"=w398:errorcluster)  [unwired: 2 in, 1 out]
          "Timed Out? 9" <- w392
          n246 = call "Tick Count9"() -> ("Tick Count(Ticks)"=w409:u8)
          n247 = feedback #13(u8 0 ("Tick Count(uSec)")) -> (w410:u8)
          n248 = feedback-in #13(w409) -> ()
          n249 = Subtract(x=w409, y=w410) -> (x-y=→"DITTL LOOP TICKS":u8)
          n250 = xnode "FPGA I/O Node"() -> ("error out"=w400:errorcluster, "Mod2/DIO0"=w405:bool, "Mod2/DIO1"=w404:bool)  [unwired: 3 in, 2 out]
          n251 = Merge Errors(w400, w399, w398) -> (w397:errorcluster)
          n252 = Unbundle By Name(w397) -> ("status"=w407:bool)
          n253 = Compound Arithmetic op=OR(w407, w393, w392) -> (w406:bool)
          n254 = case shown="True" w406 {
            selector: w406 -> [_ w413]
            tunnel: [FALSE w413] -> w396
            frame False {
            }
            frame True {
              n255 = local write "StopLoops"(w413) -> ()
            }
          }
          n256 = local read "StopLoops"() -> (w394:bool)
          n257 = call "Loop Timer"("Count(Ticks)"="TTL sample period (ticks)") -> ()  [unwired: 1 out]
          n258 = Or(x=w396, y=w394) -> (x .or. y?=w395:bool)
        }
        n259 = while {
          tunnel: [w421] -> w353
          stop <- w417 stop-if-true
          # "1MS/s 24V digital write"
          n260 = feedback #14(u32 0 ("State machine iterations")) -> (w415:u32)
          n261 = call "Tick Count8"() -> ("Tick Count(Ticks)"=w424:u8)
          n262 = Increment(x=w415) -> (x+1=w414:u32)
          "DO24V" <- w414
          n263 = feedback-in #14(w414) -> ()
          n264 = feedback #15(u8 0 ("Tick Count(uSec)")) -> (w425:u8)
          n265 = feedback-in #15(w424) -> ()
          n266 = Subtract(x=w424, y=w425) -> (x-y=→"FBI LOOP TICKS":u8)
          n267 = xnode ("FIFO Method Node")("Timeout"=40) -> ("Element"=w429:bool, "Timed Out?"=w427:bool, "error out"=w428:errorcluster)  [unwired: 2 in, 1 out]
          "Timed Out? 8" <- w427
          n268 = case shown="False" w427 {
            tunnel: w429 -> [w434 _]
            tunnel: [w433 _] -> w421
            frame False {
              n269 = xnode "FPGA I/O Node"("Mod4/DO0"=w434) -> ("error out"=w433:errorcluster)  [unwired: 2 in, 1 out]
            }
            frame True {
            }
          }
          n270 = Merge Errors(w421, w428) -> (w422:errorcluster)
          n271 = Unbundle By Name(w422) -> ("status"=w420:bool)
          n272 = case shown="True" w420 {
            selector: w420 -> [_ w432]
            tunnel: [FALSE w432] -> w419
            frame False {
            }
            frame True {
              n273 = local write "StopLoops"(w432) -> ()
            }
          }
          n274 = local read "StopLoops"() -> (w418:bool)
          n275 = Or(x=w419, y=w418) -> (x .or. y?=w417:bool)
        }
        n276 = while {
          shift-right: [w441] -> w358
          shift-left: _ -> [w460]
          shift-right: [w456] -> _
          shift-left: _ -> [w459]
          shift-right: [w457] -> _
          shift-left: _ -> [w458]
          stop <- w444 stop-if-true
          w453 = 0 ("Timeout")
          n277 = feedback #16(u32 0 ("State machine iterations")) -> (w436:u32)
          n278 = Increment(x=w436) -> (x+1=w435:u32)
          "AQ ANALOG AI01" <- w435
          n279 = feedback-in #16(w435) -> ()
          n280 = xnode ("FIFO Method Node")("Element"=w459, "Timeout"=w453, "error in (no error)"=w460) -> ("Timed Out?"=w439:bool, "error out"=w455:errorcluster)  [unwired: 1 in, 1 out]
          "Timed Out?" <- w439
          n281 = xnode ("FIFO Method Node")("Element"=w458, "Timeout"=w453) -> ("Timed Out?"=w438:bool, "error out"=w454:errorcluster)  [unwired: 2 in, 1 out]
          "Timed Out? 2" <- w438
          n282 = call "Tick Count11"() -> ("Tick Count(Ticks)"=w449:u8)
          n283 = feedback #17(u8 0 ("Tick Count(uSec)")) -> (w450:u8)
          n284 = feedback-in #17(w449) -> ()
          n285 = Subtract(x=w449, y=w450) -> (x-y=→"ANALOG LOOP TICKS 2":u8)
          n286 = xnode "Read I/O Method"("Timeout"="AI Timeout") -> ("error out"=w442:errorcluster, "Mod1/AI0"=w456:fxp<+/-,24,5>, "Mod1/AI1"=w457:fxp<+/-,24,5>, "Timed Out"=w443:bool)  [unwired: 3 in, 2 out]
          "A. READ timeout" <- w443
          n287 = Merge Errors(w442, w455, w454) -> (w441:errorcluster)
          n288 = Unbundle By Name(w441) -> ("status"=w440:bool)
          n289 = Compound Arithmetic op=OR(w443, w440, w439, w438) -> (w447:bool)
          n290 = case shown="True" w447 {
            selector: w447 -> [_ w462]
            tunnel: [FALSE w462] -> w446
            frame False {
            }
            frame True {
              n291 = local write "StopLoops"(w462) -> ()
            }
          }
          n292 = local read "StopLoops"() -> (w445:bool)
          n293 = Or(x=w446, y=w445) -> (x .or. y?=w444:bool)
        }
        n294 = while {
          tunnel: [w582] -> w356
          tunnel: "AI sample period (usec)" -> [w581]
          stop <- w574 stop-if-true
          n295 = flat-sequence {
            tunnel: w581 -> [w585]
            tunnel: [w588] -> w582
            tunnel: [w587] -> w579
            tunnel: [w586] -> w578
            frame #0 {
              n296 = call "Loop Timer4"("Count(uSec)"=w585) -> ()  [unwired: 1 out]
            }
            frame #1 {
              n297 = xnode "Get I/O Read Status Method"() -> ("error out"=w588:errorcluster, "Overwrite"=w587:bool, "Sample Gated"=w586:bool)  [unwired: 3 in, 2 out]
            }
          }
          n298 = feedback #18(u32 0 ("State machine iterations")) -> (w572:u32)
          n299 = Increment(x=w572) -> (x+1=w571:u32)
          "AQ ANALOG STATUS" <- w571
          n300 = feedback-in #18(w571) -> ()
          n301 = Unbundle By Name(w582) -> ("status"=w580:bool)
          n302 = Compound Arithmetic op=OR(w580, w579, w578) -> (w577:bool)
          n303 = case shown="True" w577 {
            selector: w577 -> [_ w584]
            tunnel: [FALSE w584] -> w576
            frame False {
            }
            frame True {
              n304 = local write "StopLoops"(w584) -> ()
            }
          }
          n305 = local read "StopLoops"() -> (w575:bool)
          n306 = Or(x=w576, y=w575) -> (x .or. y?=w574:bool)
          "Overwrite" <- w579
          "Sample Gated" <- w578
        }
        n307 = Merge Errors(w356, w357, w358, w354, w352, w353) -> (→"Read/write Error":errorcluster)
      }
    }
    "BULCE AQ GRANDE" <- w339
  }
  "Duty & Pulse OK?" <- TRUE ("Duty & Pulse OK?")
  "FBI" <- TRUE ("FBI")
  "SRCDuty" <- fxp<+,32,32> 20.0 ("maxDuty")
  "SRCPulse" <- u32 120200 ("maxHigh")
